vi "[ex ce] 2 Obtaining result via variables.vi"() -> ()   [LabVIEW 2021]
doc: "<B>Obtaining results via variables</B> (CE Client Example)\n\nThis simple example demonstrates how you can use CalcExpress for remote computation and obtain results via variables. Similar to this example, you can obtain results of any type supported by CalcExpress.\n\nTo execute this example, you need run <B>[ex ce] CE Server Example.vi</B> on either local or remote computer. Also, you need the <B>LabVIEW Advanced Analysis VIs</B> on server side.\n\n::: CalcExpress Toolkit :::\nCopyright (c) 2000-2026 Konstantin Shifershteyn. All rights reserved."
panel:
  out "dbl result":dbl caption="dbl result. It's value of mean(z) for this example script" format="%.3f"
  in  "To execute this example, you need run the \"[ex ce] CE Server Example.vi\" on either local or remote computer. Also, you need the Advanced Analysis Libraries on server side.\n-------------------------------------------\nThis simple example demonstrates how you can use CalcExpress for remote computation and obtain results via variables. Similar to this example, you can obtain results of any type supported by CalcExpress.":string="To execute this example, you need run the \"[ex ce] CE Server Example.vi\" on either local or remote computer. Also, you need the Advanced Analysis Libraries on server side.\n-------------------------------------------\nThis simple example demonstrates how you can use CalcExpress for remote computation and obtain results via variables. Similar to this example, you can obtain results of any type supported by CalcExpress."
  in  "results list":string="x\ny\nz"
  in  "use TCP for local":bool
  in  "expression":string="x = pPulse(1000, 2, 200, 400); //pulse pattern\ny = pSine (1000, 1, 0, 5 );    //sine pattern\nz = abs(x*y);\nmean(z)"
  out "graph":dbl[][](graph)
  in  "port":u32=3363
  in  "machine name (empty - local)":string
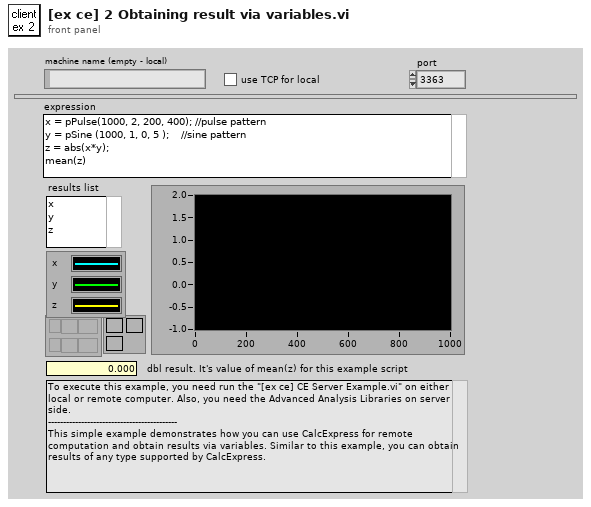
[diagram p1: front panel]
types:
  T1 = typedef "CE Session.ctl" = cluster{"VI refnum":refnum<vi>, "VC Handle":T2}
  T2 = typedef "VarMan Variable Context Handle.ctl" = i32
  T3 = typedef "CalcExpress Data Type.ctl" = enum32{"String", "DBL Number", "identifier", "1D Array of DBL", "2D Array of DBL", "CDB Number", "1D Array of CDB", "2D Array of CDB", "1D Array of String", "2D Array of String", "Unknown data type"}
  T4 = cluster{"type":T3, "dbl":dbl, "cdb":cdb, "str":string, "1d dbl":dbl[], "1d cdb":cdb[], "1d str":string[], "2d dbl":dbl[][], "2d cdb":cdb[][], "2d str":string[][]}
  T5 = enum16{"create", "destroy", "set value", "get value"}
  T6 = enum32{"String", "DBL Number", "identifier", "1D Array of DBL", "2D Array of DBL", "CDB Number", "1D Array of CDB", "2D Array of CDB", "1D Array of String", "2D Array of String", "Unknown data type"}
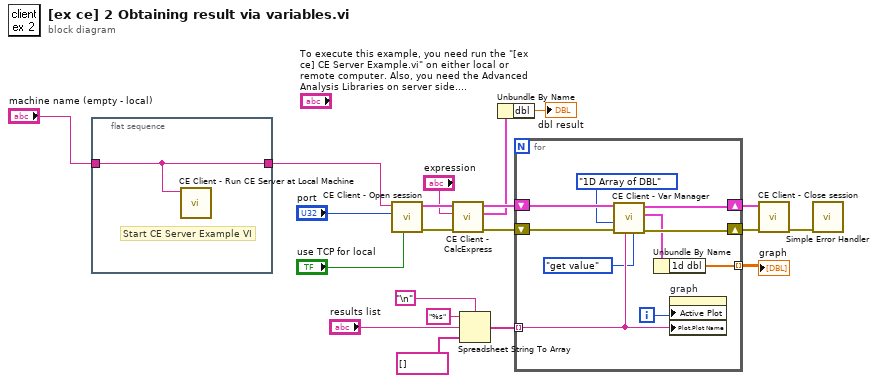
[diagram p0: block diagram]
diagram:
  n1 = flat-sequence {
    tunnel: [w21] -> w7
    tunnel: "machine name (empty - local)" -> [w21]
    frame #0 {
      # "Start CE Server Example VI"
      n2 = call "CE Client - Run CE Server at Local Machine.vi"("machine name"=w21) -> ()  [unwired: 9 in, 2 out]
    }
  }
  n3 = call "CE Client - Open session.vi"("use TCP for local (F)"="use TCP for local", "port number (3363)"="port", "machine name (empty - local)"=w7) -> ("error out"=w19:errorcluster, "CE session out"=w20:T1)  [unwired: 5 in]
  n4 = call "CE Client - CalcExpress.vi"("error in"=w19, "expression"="expression", "CE session"=w20) -> ("error out"=w14:errorcluster, "values out"=w8:T4, "dup CE session"=w12:T1)  [unwired: 4 in]
  n5 = Spreadsheet String To Array(delimiter (Tab)="\n", format string="%s", spreadsheet string="results list", array type (2D Dbl)=string[] [] ("Array out")) -> (array=w2:string[])
  n6 = Unbundle By Name(w8) -> ("dbl"=→"dbl result":dbl)
  n7 = for {
    shift-right: [w28] -> w13
    shift-left: w14 -> [w31]
    shift-right: [w29] -> w10
    shift-left: w12 -> [w30]
    tunnel: [w27] -> w11 mode=indexing
    tunnel: w2 -> [w25] mode=indexing
    i -> [w26]
    n8 = call "CE Client - Var Manager.vi"("var cmd"=T5."get value", "var name"=w25, "error in"=w31, "var type"=T6."1D Array of DBL" ("data type"), "CE session"=w30) -> ("error out"=w28:errorcluster, "values out"=w23:T4, "dup CE session"=w29:T1)  [unwired: 2 in]
    n9 = Unbundle By Name(w23) -> ("1d dbl"=w27:dbl[])
    n10 = property on="graph" class="WFGraph (strict)"("Active Plot"=w26, "Plot.Plot Name"=w25) -> ()  [unwired: 2 in, 2 out]
  }
  "graph" <- w11
  n11 = call "CE Client - Close session.vi"("error in"=w13, "CE session"=w10) -> ("error out"=w17:errorcluster)  [unwired: 6 in, 1 out]
  n12 = call <vilib>:"Simple Error Handler.vi"("error in (no error)"=w17) -> ()  [unwired: 4 in, 5 out]
